vi "DeleteDC Wrapper Template.vi"(0 "hdc":u64, 11 "error in":errorcluster) -> (4 "return value":i32, 15 "error out":errorcluster)   [LabVIEW 2020]
doc: "Deletes a device context created with gdi32 CreateCompatibleDC.vi, through gdi32.dll DeleteDC (stdcall, called in any thread). Do not use it on a DC from GetDC - release that with user32 ReleaseDC.vi. return value is non-zero on success. When error in carries an error the DLL is not called. Generated by tools\\Build Win32 Wrappers.vi - do not edit by hand, rebuild it."
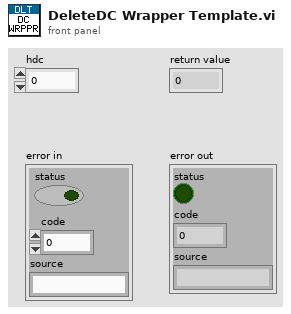
[diagram p1: front panel]
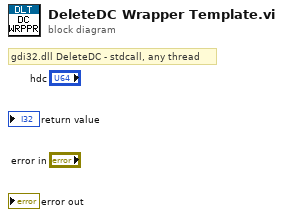
[diagram p0: block diagram]
diagram:
  # "gdi32.dll DeleteDC - stdcall, any thread"
